vi "wiringPiSPIxClose.vi"(8 "error in (no error)":errorcluster, 11 "SPI Device":T1) -> (0 "error out":errorcluster, 2 "return":i32, 3 "SPI Device out":T1)   [LabVIEW 2025, in "wiringPi.lvlib"]
doc: "<b>_______________________________________________________________</b>\n** Author: Juan José Villacorta\n** LabVIEW wrapper for C library <b> wiringPi </b>,\n** https://github.com/WiringPi/WiringPi\n<b>_______________________________________________________________</b>\n\n/*\n * wiringPiSPISetupMode:\n * Close the SPI device\n *********************************************************************************\n */"
uses:
  wiringPi.lvlib
  Type Defs/SPI Device.ctl
  Type Defs/SPI Dev.ctl
  Type Defs/SPI Channel.ctl
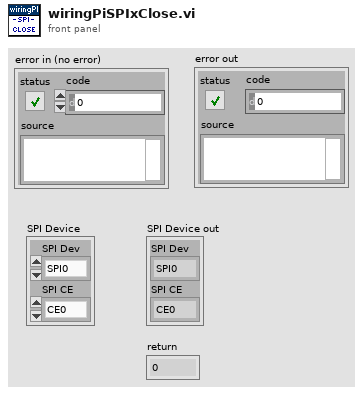
[diagram p1: front panel]
types:
  T1 = typedef "wiringPi.lvlib/SPI Device.ctl" = cluster{"SPI Dev":T2, "SPI CE":T3}
  T2 = typedef "wiringPi.lvlib/SPI Dev.ctl" = enum32{"SPI0", "SPI1"}
  T3 = typedef "wiringPi.lvlib/SPI Channel.ctl" = enum32{"CE0", "CE1", "CE2"}
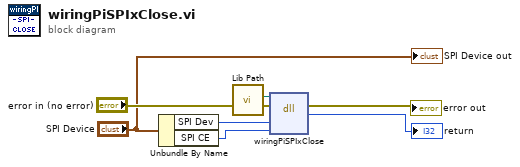
[diagram p0: block diagram]
diagram:
  n1 = Unbundle By Name("SPI Device") -> ("SPI Dev"=w5:T2, "SPI CE"=w4:T3)
  n2 = call "Lib Path.vi"() -> ("path out"=w1:path)  [unwired: 11 in]
  n3 = dll-call lib="libLVwiringPI.so" fn="wiringPiSPIxClose"(path in=w1, error in="error in (no error)", "number"=w5, "channel"=w4) -> (error out=→"error out":errorcluster, "return type"=→"return":i32)  [unwired: 3 in, 1 out]
  "SPI Device out" <- "SPI Device"
